vi "SPARK Configure Alt Ext Encoder.vi"   [LabVIEW 2027]
doc: "Configure the alternate or external encoder connected to the data port of the SPARK."
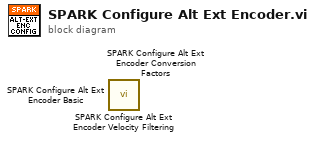
[diagram p0: block diagram]
diagram:
  n1 = call <vilib>:"SPARK Configure Alt Ext Encoder Velocity Filtering.vi"() -> ()  [unwired: 10 in, 2 out]
  n2 = call <vilib>:"SPARK Configure Alt Ext Encoder Conversion Factors.vi"() -> ()  [unwired: 10 in, 2 out]
  n3 = call <vilib>:"SPARK Configure Alt Ext Encoder Basic.vi"() -> ()  [unwired: 10 in, 2 out]
